vi "PhotonCamera_GetLEDMode.vi"(11 "BaseNTName":string="/photonvision") -> (0 "error out":errorcluster, 3 "LEDMode":T1)   [LabVIEW 2019, in "PhotonVisionLib.lvlib"]
doc: "Returns the current LED mode.\n\nInputs:\n - BaseNTName - string - Base Nework Table name. (Optional. Default: /photonvision )\n\nOutputs:\n - LedMode -- The current LED mode.\n - Error Out -- Contains error information if a Network table ot other error occured."
uses:
  PhotonVisionLib.lvlib
  Enum/VisionLEDModeType.ctl
  <vilib>/Rock Robotics/Network Tables/NT Read Integer.vi
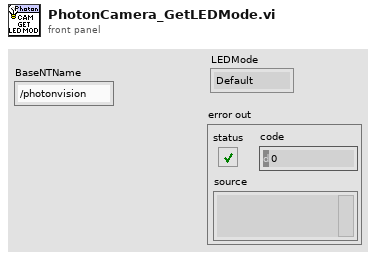
[diagram p1: front panel]
types:
  T1 = typedef "PhotonVisionLib.lvlib/VisionLEDModeType.ctl" = enum16{"Default", "Off", "On", "Blink"}
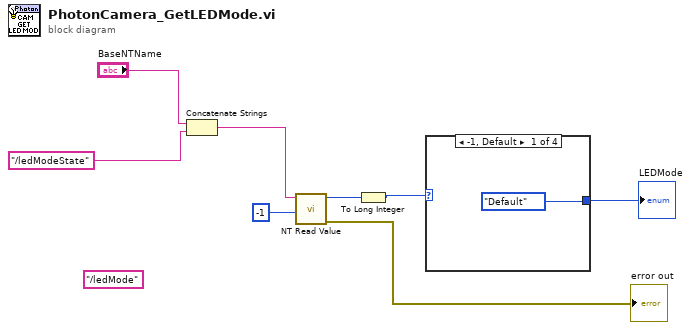
[diagram p0: block diagram]
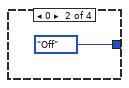
[diagram p2: hidden frame]
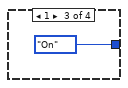
[diagram p3: hidden frame]
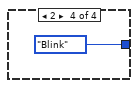
[diagram p4: hidden frame]
diagram:
  (unwired) "/ledMode"
  n1 = Concatenate Strings("BaseNTName", "/ledModeState") -> (w1:string)
  n2 = call-poly <vilib>:"NT Read Value.vi"("default value"=i64 -1 ("Default Value"), "name"=w1) -> ("error out"=→"error out":errorcluster, "value"=w7:i64)  [unwired: 7 in, 1 out]
  n3 = To Long Integer(number=w7) -> (32bit integer=w6:i32)
  n4 = case shown="-1, Default" w6 {
    tunnel: [VisionLEDModeType."Default" ("LEDMode") VisionLEDModeType."Off" ("LEDMode") VisionLEDModeType."On" ("LEDMode") VisionLEDModeType."Blink" ("LEDMode")] -> w5
    frame -1, Default {
    }
    frame 0 {
    }
    frame 1 {
    }
    frame 2 {
    }
  }
  "LEDMode" <- w5
